vi "LB_AssertAllItems_Tests.vi"(11 "error in":errorcluster) -> (15 "error out":errorcluster)   [LabVIEW 2016, in "DronaTest.lvlib"]
uses:
  DronaTest.lvlib
  APIs/Stimulus/ControlValue/SetValueAuto.vi
  APIs/Assert/AssertControlValue/Controls/Listbox/AssertAllItems.vi
  <vilib>/addons/_JKI Toolkits/Caraya/classes/Assert/Assert Error.vi
  <vilib>/addons/_JKI Toolkits/Caraya/classes/Assert/Assert Equal Value_Variant.vi
  <vilib>/addons/_JKI Toolkits/Caraya/classes/Test/Test.lvclass
  Drona.lvlib
  <vilib>/SLL Toolkit/SLL Debug/SLL Debug.lvlib
  <vilib>/addons/_JKI Toolkits/Caraya/classes/Assert/Assert.lvclass
  APIs/Assert/AssertControlValue/Controls/Listbox/AssertListbox.lvlib
  APIs/Stimulus/ControlValue/ControlValue.lvlib
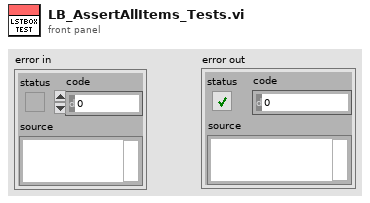
[diagram p1: front panel]
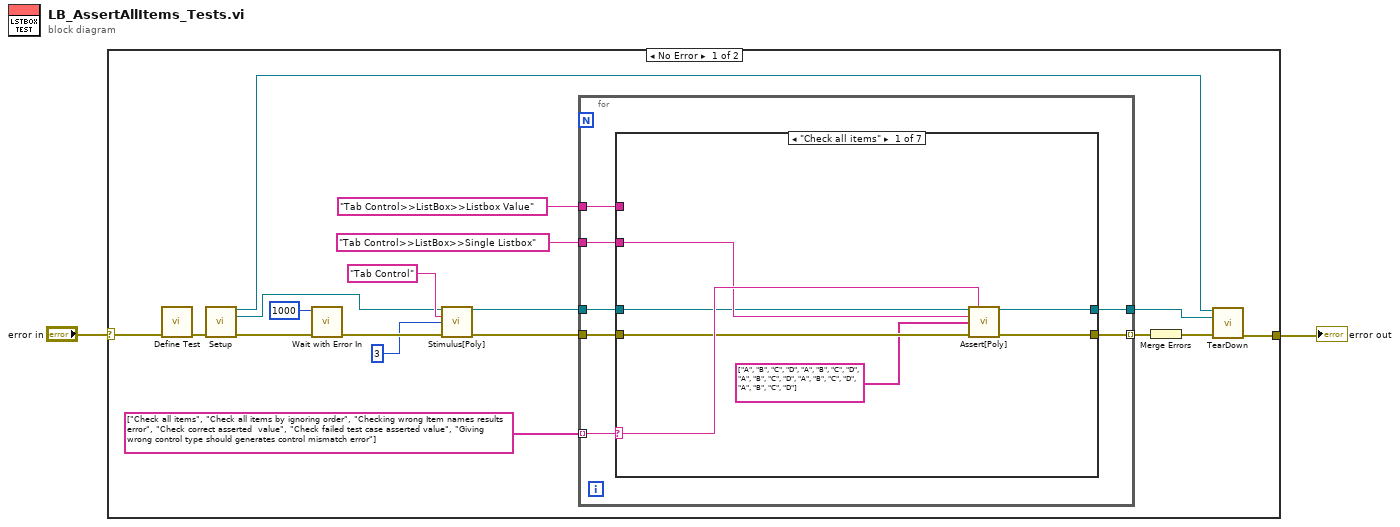
[diagram p0: block diagram]
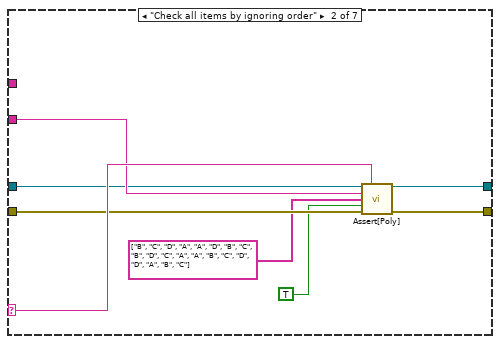
[diagram p2: hidden frame]
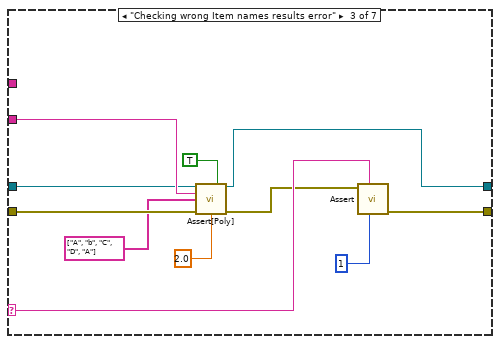
[diagram p3: hidden frame]
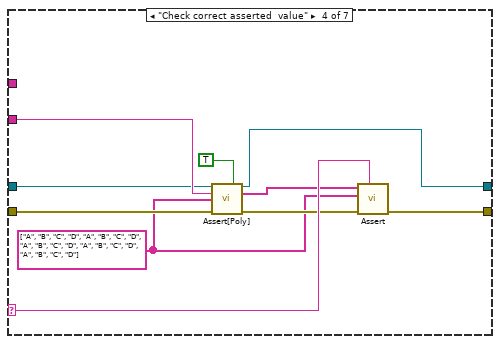
[diagram p4: hidden frame]
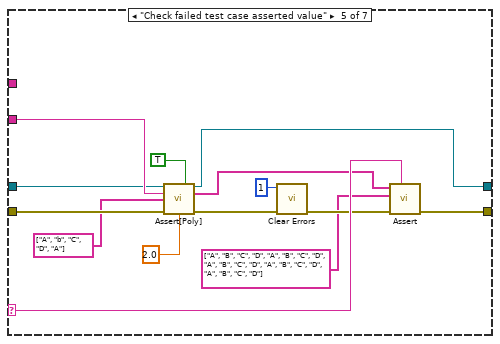
[diagram p5: hidden frame]
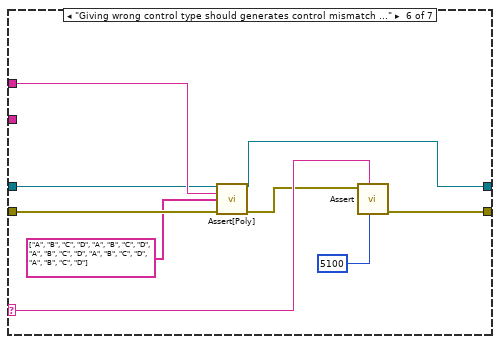
[diagram p6: hidden frame]
diagram:
  n1 = case shown="No Error" "error in" {
    selector: "error in" -> [w20 w89]
    tunnel: [w3 w89] -> w1
    frame No Error {
      n2 = call <vilib>:"Define Test.vi"("error in (no error)"=w20) -> ("error out"=w9:errorcluster)  [unwired: 9 in, 1 out]
      n3 = call "Setup.vi"("error in"=w9) -> ("Application Ref"=w5:refnum<vi>, "VI out"=w7:refnum<vi>, "error out"=w8:errorcluster)  [unwired: 12 in]
      n4 = call <vilib>:"Wait with Error In.vi"("error in (no error)"=w8, "milliseconds to wait"=u32 1000) -> ("error out"=w18:errorcluster)  [unwired: 9 in]
      n5 = call-poly "Stimulus[Poly].vi"("VI Reference In"=w7, "Control Path"="Tab Control", "Value (Signaling)"=3, "error in"=w18) -> ("VI Reference Out"=w14:refnum<vi>, "error out"=w17:errorcluster)  [unwired: 10 in]
      n6 = for {
        tunnel: w14 -> [w26]
        tunnel: "Tab Control>>ListBox>>Single Listbox" ("Control Path") -> [w25]
        tunnel: "Tab Control>>ListBox>>Listbox Value" ("Control Path") -> [w24]
        tunnel: string[] ["Check all items", "Check all items by ignoring order", "Checking wrong Item names results error", "Check correct asserted  value", "Check failed test case asserted value", "Giving wrong control type should generates control mismatch error"] -> [w22] mode=indexing
        tunnel: [w21] -> w4
        tunnel: w17 -> [w27]
        tunnel: [w23] -> w10 mode=indexing
        n7 = case shown="\"Check all items\"" w22 {
          selector: w22 -> [w32 w40 w52 w62 w76 w85 _]
          tunnel: w27 -> [w30 w38 w45 w58 w72 w80 w88]
          tunnel: w26 -> [w29 w37 w44 w57 w71 w79 w87]
          tunnel: w25 -> [w31 w39 w50 w61 w75 _ _]
          tunnel: w24 -> [_ _ _ _ _ w82 _]
          tunnel: [w34 w42 w53 w63 w77 w86 w88] -> w23
          tunnel: [w33 w41 w49 w60 w74 w81 w87] -> w21
          frame "Check all items" {
            n8 = call-poly "Assert[Poly].vi"("VI Reference In"=w29, "Test Label"=w32, "Control Path"=w31, "Item Names"=string[] ["A", "B", "C", "D", "A", "B", "C", "D", "A", "B", "C", "D", "A", "B", "C", "D", "A", "B", "C", "D"], "Error In"=w30) -> ("VI Reference Out"=w33:refnum<vi>, "Error Out"=w34:errorcluster)  [unwired: 8 in, 1 out]
          }
          frame "Check all items by ignoring order" {
            n9 = call-poly "Assert[Poly].vi"("VI Reference In"=w37, "Test Label"=w40, "Control Path"=w39, "Item Names"=string[] ["B", "C", "D", "A", "A", "D", "B", "C", "B", "D", "C", "A", "A", "B", "C", "D", "D", "A", "B", "C"], "Ignore Order? (F)"=TRUE, "Error In"=w38) -> ("VI Reference Out"=w41:refnum<vi>, "Error Out"=w42:errorcluster)  [unwired: 7 in, 1 out]
          }
          frame "Checking wrong Item names results error" {
            n10 = call-poly "Assert[Poly].vi"("VI Reference In"=w44, "Assert Only? (F)"=TRUE, "Control Path"=w50, "Item Names"=string[] ["A", "b", "C", "D", "A"], "Error In"=w45, "Timeout(5 sec)"=2.0) -> ("VI Reference Out"=w49:refnum<vi>, "Error Out"=w48:errorcluster)  [unwired: 7 in, 1 out]
            n11 = call-poly <vilib>:"Assert.vi"("error code (1)"=1, "Label"=w52, "Error?"=w48) -> ("error out"=w53:errorcluster)  [unwired: 7 in, 1 out]
          }
          frame "Check correct asserted  value" {
            w54 = string[] ["A", "B", "C", "D", "A", "B", "C", "D", "A", "B", "C", "D", "A", "B", "C", "D", "A", "B", "C", "D"] ("Item Names")
            n12 = call-poly "Assert[Poly].vi"("VI Reference In"=w57, "Assert Only? (F)"=TRUE, "Control Path"=w61, "Item Names"=w54, "Error In"=w58) -> ("VI Reference Out"=w60:refnum<vi>, "Asserted Value"=w55:string[], "Error Out"=w56:errorcluster)  [unwired: 8 in]
            n13 = call-poly <vilib>:"Assert.vi"("Label"=w62, "error in (no error)"=w56, "Y"=w54, "X"=w55) -> ("error out"=w63:errorcluster)  [unwired: 6 in, 1 out]
          }
          frame "Check failed test case asserted value" {
            n14 = call-poly "Assert[Poly].vi"("VI Reference In"=w71, "Assert Only? (F)"=TRUE, "Control Path"=w75, "Item Names"=string[] ["A", "b", "C", "D", "A"], "Error In"=w72, "Timeout(5 sec)"=2.0) -> ("VI Reference Out"=w74:refnum<vi>, "Asserted Value"=w69:string[], "Error Out"=w70:errorcluster)  [unwired: 7 in]
            n15 = call <vilib>:"Clear Errors.vi"("error in (no error)"=w70, "specific error code to clear (0: all)"=1) -> ("error out"=w68:errorcluster)  [unwired: 4 in, 1 out]
            n16 = call-poly <vilib>:"Assert.vi"("Label"=w76, "error in (no error)"=w68, "Y"=string[] ["A", "B", "C", "D", "A", "B", "C", "D", "A", "B", "C", "D", "A", "B", "C", "D", "A", "B", "C", "D"] ("Item Names"), "X"=w69) -> ("error out"=w77:errorcluster)  [unwired: 6 in, 1 out]
          }
          frame "Giving wrong control type should generates control mismatch error" {
            n17 = call-poly "Assert[Poly].vi"("VI Reference In"=w79, "Control Path"=w82, "Item Names"=string[] ["A", "B", "C", "D", "A", "B", "C", "D", "A", "B", "C", "D", "A", "B", "C", "D", "A", "B", "C", "D"], "Error In"=w80) -> ("VI Reference Out"=w81:refnum<vi>, "Error Out"=w83:errorcluster)  [unwired: 9 in, 1 out]
            n18 = call-poly <vilib>:"Assert.vi"("error code (1)"=5100, "Label"=w85, "Error?"=w83) -> ("error out"=w86:errorcluster)  [unwired: 7 in, 1 out]
          }
          frame Default {
          }
        }
      }
      n19 = Merge Errors(w10) -> (w6:errorcluster)
      n20 = call "TearDown.vi"("Application Ref"=w5, "VI in"=w4, "error in (no error)"=w6) -> ("error out"=w3:errorcluster)  [unwired: 12 in]
    }
    frame Error {
    }
  }
  "error out" <- w1
